vi "update listbox Items.vi"(7 "Unicode?":bool, 8 "error in (no error)":errorcluster, 10 "Data[]":string[](array[string]), 11 "Listbox Ref":refnum<vi>) -> (0 "error out":errorcluster, 3 "Listbox Ref":refnum<vi>)   [LabVIEW 2019, in "Language Selection.lvlib"]
doc: "Uses \"Data[]\" input array to translate a Listbox control items.\n- - -\nCopyright (c) 2026, Merecs Engineering GmbH"
uses:
  Language Selection.lvlib
panel:
  # "Connector Pane"
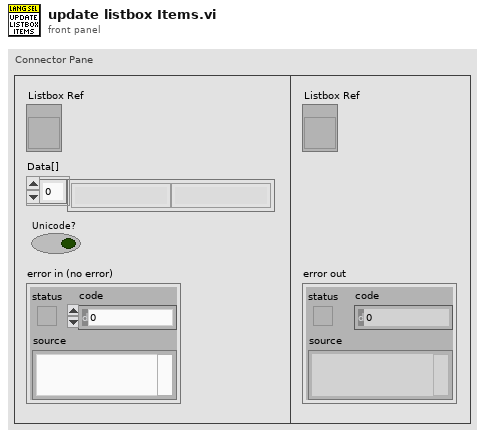
[diagram p1: front panel]
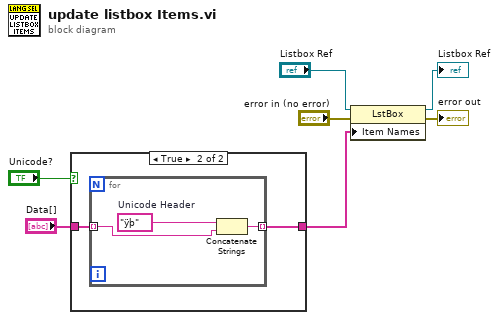
[diagram p0: block diagram]
diagram:
  n1 = case shown="True" "Unicode?" {
    tunnel: "Data[]" -> [w8 w10]
    tunnel: [w8 w9] -> w6
    frame False {
    }
    frame True {
      n2 = for {
        tunnel: w10 -> [w13] mode=indexing
        tunnel: [w12] -> w9 mode=indexing
        w11 = "ÿþ"  # Unicode Header
        n3 = Concatenate Strings(w11, w13) -> (w12:string)
      }
    }
  }
  n4 = property class="LstBox"(reference="Listbox Ref", error in="error in (no error)", "Item Names"=w6) -> (reference out=→"Listbox Ref":refnum<vi>, error out=→"error out":errorcluster)
